vi "Measure the Function on 2nd Display.vi"(7 "Manual Range":dbl format="%#.9e", 8 "error in":errorcluster, 9 "Enable Auto Range":bool=TRUE, 10 "Function":u8(ring) items=["DC Voltage", "AC Voltage", "DC Current", "AC Current", "2-Wire Resistance", "4-Wire Resistance", "Frequency", "Period"], 11 "VISA resource name":refnum<visa-resource-name>) -> (0 "error out":errorcluster, 2 "Return the Value":string, 3 "VISA resource name out":refnum<visa-resource-name>)   [LabVIEW 2012, in "GDM-9052.lvlib"]
uses:
  GDM-9052.lvlib
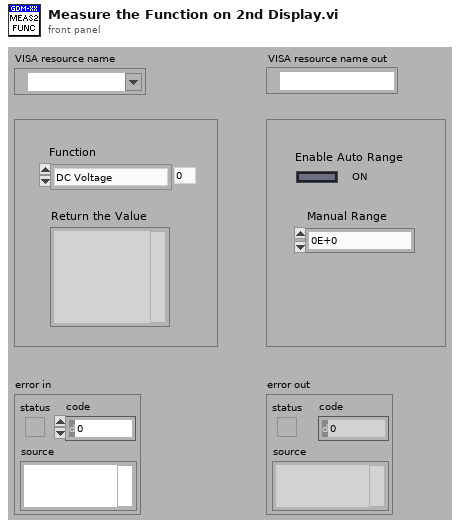
[diagram p1: front panel]
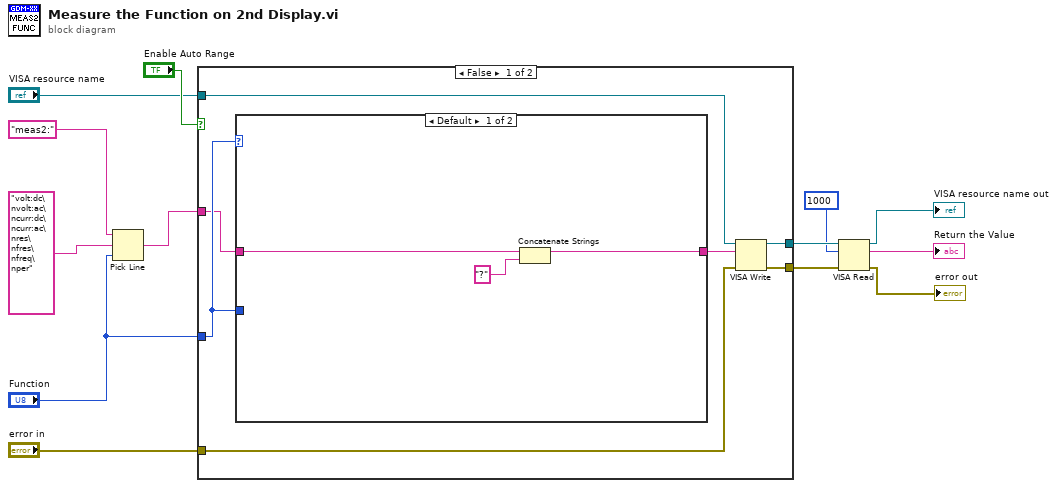
[diagram p0: block diagram]
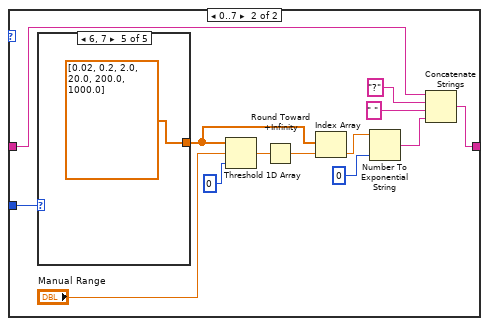
[diagram p2: hidden frame]
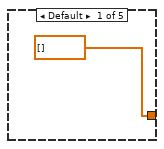
[diagram p3: hidden frame]
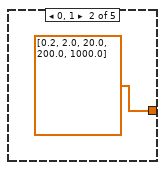
[diagram p4: hidden frame]
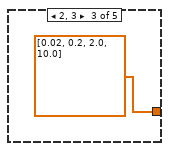
[diagram p5: hidden frame]
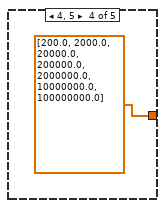
[diagram p6: hidden frame]
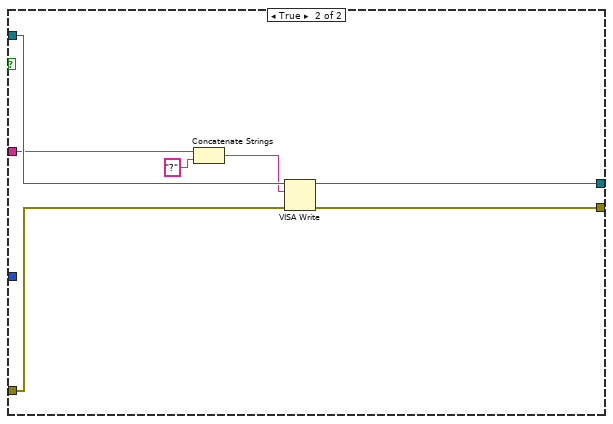
[diagram p7: hidden frame]
diagram:
  n1 = Pick Line(string ("")="meas2:", multi-line string="volt:dc\nvolt:ac\ncurr:dc\ncurr:ac\nres\nfres\nfreq\nper", line index="Function") -> (output string=w9:string)
  n2 = case shown="False" "Enable Auto Range" {
    tunnel: "Function" -> [w20 _]
    tunnel: w9 -> [w19 w43]
    tunnel: "VISA resource name" -> [w17 w48]
    tunnel: "error in" -> [w16 w47]
    tunnel: [w15 w46] -> w6
    tunnel: [w14 w45] -> w5
    frame False {
      n3 = case shown="Default" w20 {
        tunnel: w20 -> [_ w27]
        tunnel: w19 -> [w22 w29]
        tunnel: [w21 w28] -> w18
        frame Default {
          n4 = Concatenate Strings(w22, "?" ("string")) -> (w21:string)
        }
        frame 0..7 {
          n5 = case shown="6, 7" w27 {
            tunnel: [dbl[] [] dbl[] [0.2, 2.0, 20.0, 200.0, 1000.0] dbl[] [0.02, 0.2, 2.0, 10.0] dbl[] [200.0, 2000.0, 20000.0, 200000.0, 2000000.0, 10000000.0, 100000000.0] dbl[] [0.02, 0.2, 2.0, 20.0, 200.0, 1000.0]] -> w32
            frame Default {
            }
            frame 0, 1 {
            }
            frame 2, 3 {
            }
            frame 4, 5 {
            }
            frame 6, 7 {
            }
          }
          n6 = Threshold 1D Array(1:0 ("start index (0)"), 2:"Manual Range", 3:w32) -> (0:w34:dbl)
          n7 = Round Toward +Infinity(x=w34) -> (ceil(x): smallest int >= x=w33:dbl)
          n8 = Index Array(array=w32, index=w33) -> (element=w31:dbl)
          n9 = Number To Exponential String(number=w31, precision (6)=i16 0) -> (E-format string=w24:string)  [unwired: 2 in]
          n10 = Concatenate Strings(w29, "?" ("string"), " " ("string"), w24) -> (w28:string)
        }
      }
      n11 = VISA Write(VISA resource name=w17, write buffer=w18, error in (no error)=w16) -> (VISA resource name out=w15:refnum<visa-resource-name>, error out=w14:errorcluster)  [unwired: 1 out]
    }
    frame True {
      n12 = Concatenate Strings(w43, "?" ("string")) -> (w42:string)
      n13 = VISA Write(VISA resource name=w48, write buffer=w42, error in (no error)=w47) -> (VISA resource name out=w46:refnum<visa-resource-name>, error out=w45:errorcluster)  [unwired: 1 out]
    }
  }
  n14 = VISA Read(VISA resource name=w6, byte count=u32 1000, error in (no error)=w5) -> (VISA resource name out=→"VISA resource name out":refnum<visa-resource-name>, read buffer=→"Return the Value":string, error out=→"error out":errorcluster)  [unwired: 1 out]
